vi "Update_Lamps.vi"(8 "error in (no error)":errorcluster, 9 "PausedNow":bool, 10 "CurrentState":T1, 11 "TCP Network Connection in":refnum<k5>) -> (0 "error out":errorcluster, 3 "connection ID out":refnum<k5>)   [LabVIEW 2018]
uses:
  07_QMH.vi/State.ctl
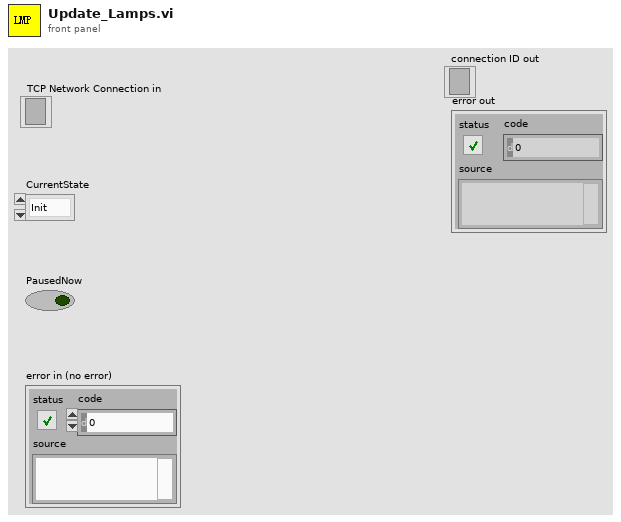
[diagram p1: front panel]
types:
  T1 = typedef "State.ctl" = enum16{"Init", "RequestPart", "WaitEntry", "WaitInPos", "WaitClamp", "Inspect", "Release", "WaitRelease", "WaitSort", "PushNG", "WaitPushExt", "WaitPushRet", "DeliverOK", "WaitExit", "WaitExitClear", "Done", "Error", "Stop", "Idle", "Pause", "Resume", "AlarmWait", "PurgeStart", "PurgeRun", "PurgePush", "PurgePushRet", "PurgeEnd"}
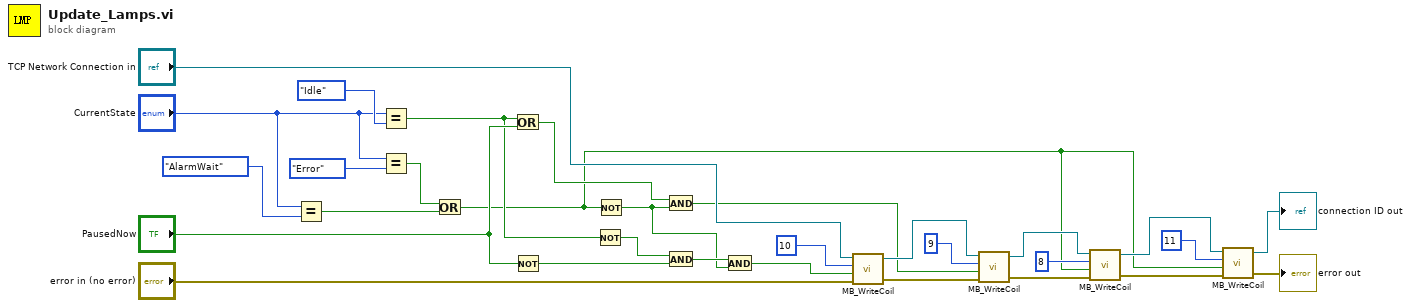
[diagram p0: block diagram]
diagram:
  n1 = Equal?(x="CurrentState", y=State."AlarmWait" ("Enum")) -> (x = y?=w15:bool)
  n2 = Equal?(x="CurrentState", y=State."Idle" ("Enum")) -> (x = y?=w22:bool)
  n3 = Equal?(x="CurrentState", y=State."Error" ("Enum")) -> (x = y?=w16:bool)
  n4 = Or(x=w16, y=w15) -> (x .or. y?=w3:bool)
  n5 = Or(x=w22, y="PausedNow") -> (x .or. y?=w12:bool)
  n6 = Not(x="PausedNow") -> (.not. x?=w27:bool)
  n7 = Not(x=w22) -> (.not. x?=w21:bool)
  n8 = Not(x=w3) -> (.not. x?=w11:bool)
  n9 = And(x=w12, y=w11) -> (x .and. y?=w10:bool)
  n10 = And(x=w21, y=w27) -> (x .and. y?=w14:bool)
  n11 = And(x=w14, y=w11) -> (x .and. y?=w13:bool)
  n12 = call "MB_WriteCoil.vi"("connection ID"="TCP Network Connection in", "Address"=u16 10, "Value"=w13, "error in (no error)"="error in (no error)") -> ("connection ID out"=w28:refnum<k5>, "error out"=w29:errorcluster)  [unwired: 2 in]
  n13 = call "MB_WriteCoil.vi"("connection ID"=w28, "Address"=u16 9, "Value"=w10, "error in (no error)"=w29) -> ("connection ID out"=w9:refnum<k5>, "error out"=w8:errorcluster)  [unwired: 2 in]
  n14 = call "MB_WriteCoil.vi"("connection ID"=w9, "Address"=u16 8, "Value"=w3, "error in (no error)"=w8) -> ("connection ID out"=w6:refnum<k5>, "error out"=w5:errorcluster)  [unwired: 2 in]
  n15 = call "MB_WriteCoil.vi"("connection ID"=w6, "Address"=u16 11, "Value"=w3, "error in (no error)"=w5) -> ("connection ID out"=→"connection ID out":refnum<k5>, "error out"=→"error out":errorcluster)  [unwired: 2 in]
